vi "Utilization.vi"() -> ()   [LabVIEW 2019]
uses:
  <vilib>/Skyline/AssetManagement/Start Utilization (Single).vi
  Asset/Asset.lvclass
  <vilib>/Skyline/AssetManagement/NI SystemLink Asset Utilization.lvclass
panel:
  out "Iteration":i32
  in  "stop":bool
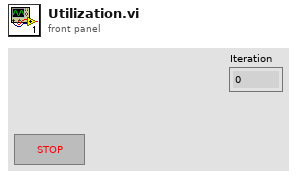
[diagram p1: front panel]
types:
  T1 = enum16{"BuiltInSystem", "PciPxi", "Usb", "Gpib", "Vxi", "Serial", "TcpIp", "cRio", "Scxi", "cDaq", "SwitchBlock", "Scc", "FireWire", "Accessory", "Can", "SwitchBlockDevice"}
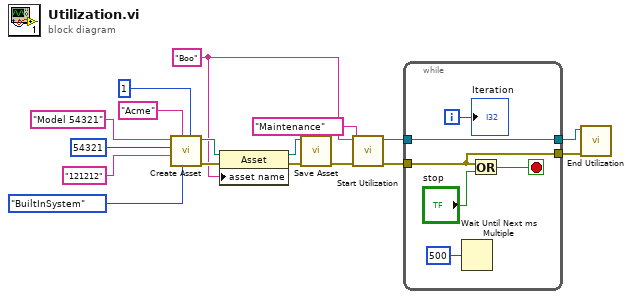
[diagram p0: block diagram]
diagram:
  w2 = "Boo" ("asset name")
  n1 = call "Create Asset.vi"("Vendor Number"=u32 1, "Bus Type"=T1."BuiltInSystem", "Vendor Name"="Acme", "Serial Number"="121212", "Model Number"=u32 54321, "Model Name"="Model 54321") -> ("Error Out"=w6:errorcluster, "Asset"=w3:refnum<class "Asset.lvclass">)  [unwired: 4 in]
  n2 = property class="Asset"(reference=w3, error in=w6, "asset name"=w2) -> (reference out=w4:refnum<class "Asset.lvclass">, error out=w5:errorcluster)
  n3 = call "Save Asset.vi"("Error In"=w5, "Asset"=w4) -> ("Error Out"=w9:errorcluster)  [unwired: 9 in]
  n4 = call-poly <vilib>:"Start Utilization.vi"("error in (no error)"=w9, "utilization category"="Maintenance", "asset name"=w2) -> ("error out"=w16:errorcluster, "asset utilization"=w17:refnum<class "NI SystemLink Asset Utilization.lvclass">)  [unwired: 7 in]
  n5 = while {
    tunnel: [w22] -> w14
    tunnel: w17 -> [w22]
    tunnel: w16 -> [w21]
    tunnel: [w21] -> w15
    i -> [w18]
    stop <- w19 stop-if-true
    n6 = Wait Until Next ms Multiple(millisecond multiple=u32 500) -> ()  [unwired: 1 out]
    n7 = Or(x=w21, y="stop") -> (x .or. y?=w19:bool)
    "Iteration" <- w18
  }
  n8 = call <vilib>:"End Utilization.vi"("error in (no error)"=w15, "asset utilization"=w14) -> ()  [unwired: 9 in, 1 out]
